vi "Exp - Error protocol.vi"(5 "InstanceRef":T1, 6 "error in":bool, 7 "cmd (def: add)":u16(ring)=1 items=["init", "add", "get"], 8 "add FuncName (T)":bool=TRUE, 9 "error message in":string) -> (0 "error out":bool, 3 "error message out":string)   [LabVIEW 2021]
doc: "<b>*** DEPRECATED ***</b>\n\nThe VI is used to declare errors in FuncVIs.\nThis VI is obsolete. Instead of it, use \"Exp-Error handler.vi\" that has more functionality.\n\nFor more information, see help for this VI.\n\n::: CalcExpress Toolkit :::\nCopyright (c) 2000-2026 Konstantin Shifershteyn. All rights reserved."
uses:
  cetypes.llb/CalcExpress Instance RefNum.ctl
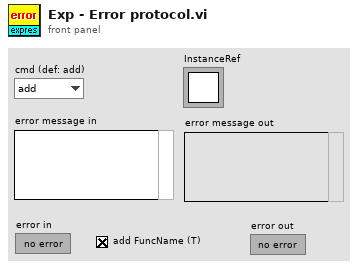
[diagram p1: front panel]
types:
  T1 = typedef "CalcExpress Instance RefNum.ctl" = refnum<k1>
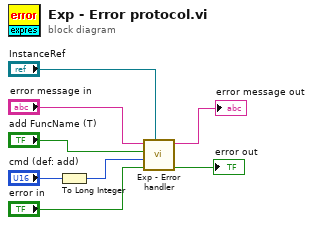
[diagram p0: block diagram]
diagram:
  n1 = To Long Integer(number="cmd (def: add)") -> (32bit integer=w1:i32)
  n2 = call "Exp - Error handler.vi"("InstanceRef"="InstanceRef", "error in"="error in", "cmd (1:set)"=w1, "add FuncName (T)"="add FuncName (T)", "error message in"="error message in") -> ("error out"=→"error out":bool, "error message out"=→"error message out":string)  [unwired: 4 in, 1 out]
